vi "ROMERO C Y ROJAS S.vi"() -> ()   [LabVIEW 2019]
uses:
  <vilib>/Instr/_visa.llb/VISA Configure Serial Port (Instr).vi
panel:
  out "read buffer":string
  in  "VISA resource name":refnum<visa-resource-name>
  in  "stop":bool
  out "LED2":bool
  out "LED1":bool
  out "Meter":dbl(knob) scale=0.0..200.0
  out "Thermometer":dbl(slide) scale=0.0..100.0
  # "VEL=125/\nTEM=80/\nLED1=ON/\nLED2=OFF/"
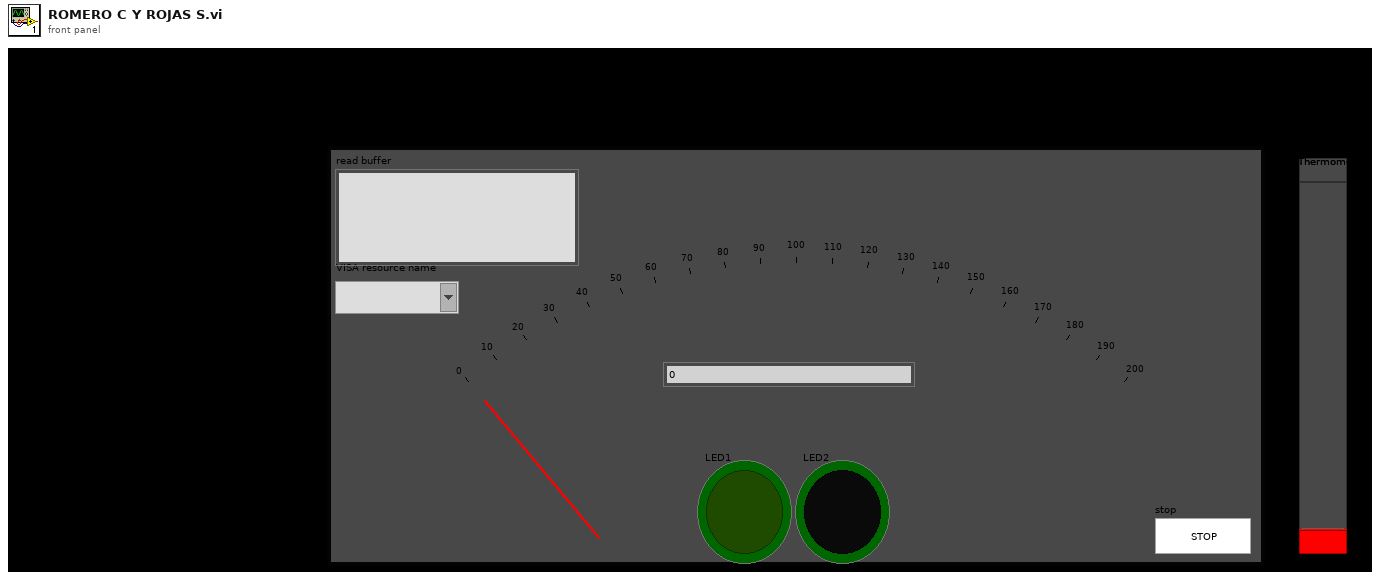
[diagram p1: front panel]
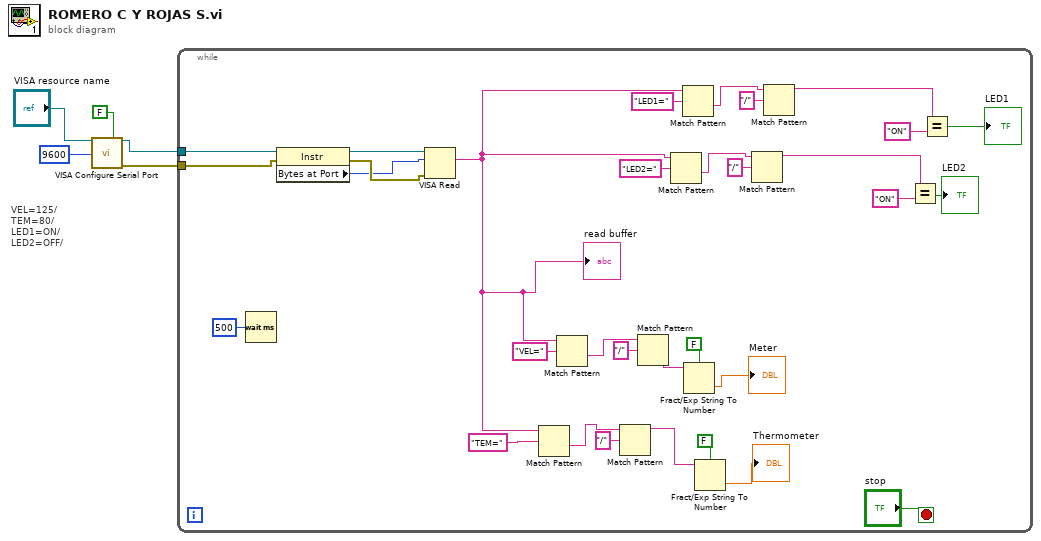
[diagram p0: block diagram]
diagram:
  # "VEL=125/\nTEM=80/\nLED1=ON/\nLED2=OFF/"
  n1 = call-poly "VISA Configure Serial Port"("VISA resource name"="VISA resource name", "Enable Termination\nChar (T)"=FALSE ("Enable Termination\nChar (T)"), "baud rate (9600)"=u32 9600) -> ("VISA resource name out"=w2:refnum<visa-resource-name>, "error out"=w1:errorcluster)  [unwired: 11 in]
  n2 = while {
    tunnel: w2 -> [w36]
    tunnel: w1 -> [w35]
    stop <- "stop" stop-if-true
    n3 = Wait (ms)(milliseconds to wait=u32 500) -> ()  [unwired: 1 out]
    n4 = property class="Instr"(reference=w36, error in=w35) -> (reference out=w33:refnum<visa-resource-name>, error out=w32:errorcluster, "Bytes at Port"=w31:u32)
    n5 = VISA Read(VISA resource name=w33, byte count=w31, error in (no error)=w32) -> (read buffer=w6:string)  [unwired: 3 out]
    "read buffer" <- w6
    n6 = Match Pattern(string=w6, regular expression="TEM=") -> (after substring=w21:string)  [unwired: 1 in, 3 out]
    n7 = Match Pattern(string=w6, regular expression="VEL=") -> (after substring=w29:string)  [unwired: 1 in, 3 out]
    n8 = Match Pattern(string=w21, regular expression="/") -> (before substring=w23:string)  [unwired: 1 in, 3 out]
    n9 = Match Pattern(string=w29, regular expression="/") -> (before substring=w27:string)  [unwired: 1 in, 3 out]
    n10 = Match Pattern(string=w6, regular expression="LED2=") -> (after substring=w10:string)  [unwired: 1 in, 3 out]
    n11 = Match Pattern(string=w6, regular expression="LED1=") -> (after substring=w16:string)  [unwired: 1 in, 3 out]
    n12 = Fract/Exp String To Number(use system decimal point (T)=FALSE, string=w27) -> (number=→"Meter":dbl)  [unwired: 2 in, 1 out]
    n13 = Fract/Exp String To Number(use system decimal point (T)=FALSE, string=w23) -> (number=→"Thermometer":dbl)  [unwired: 2 in, 1 out]
    n14 = Match Pattern(string=w10, regular expression="/") -> (before substring=w11:string)  [unwired: 1 in, 3 out]
    n15 = Match Pattern(string=w16, regular expression="/") -> (before substring=w14:string)  [unwired: 1 in, 3 out]
    n16 = Equal?(x=w11, y="ON") -> (x = y?=→"LED2":bool)
    n17 = Equal?(x=w14, y="ON") -> (x = y?=→"LED1":bool)
  }
